vi "work1_Takeorder_and_Cook.vi"() -> ()   [LabVIEW 2026]
panel:
  out "Client Served":i32
  out "element":i32
  in  "stop":bool
  in  "Order ID":i32
  # "Producer Consumer Demo"
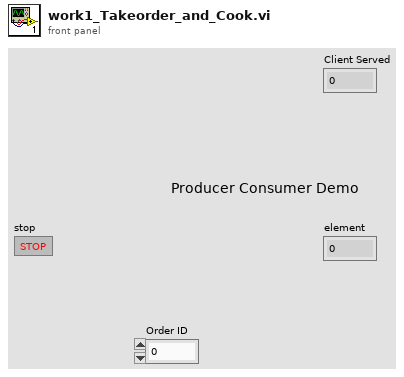
[diagram p1: front panel]
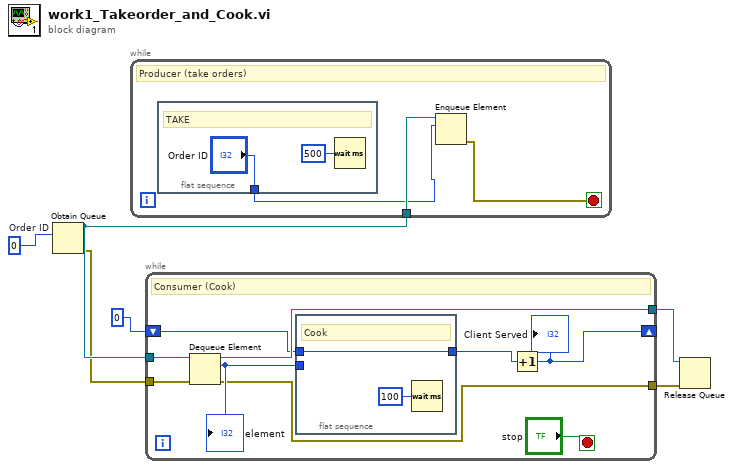
[diagram p0: block diagram]
diagram:
  w6 = 0  # Order ID
  n1 = Obtain Queue(element data type=w6) -> (queue out=w5:refnum<queue>, error out=w4:errorcluster)  [unwired: 4 in, 1 out]
  n2 = while {
    tunnel: w5 -> [w9]
    stop <- w7 stop-if-true
    # "Producer (take orders)"
    n3 = flat-sequence {
      tunnel: ["Order ID"] -> w8
      frame #0 {
        # "TAKE"
        n4 = Wait (ms)(milliseconds to wait=u32 500) -> ()  [unwired: 1 out]
      }
    }
    n5 = Enqueue Element(queue=w9, element=w8) -> (error out=w7:errorcluster)  [unwired: 2 in, 2 out]
  }
  n6 = while {
    tunnel: w5 -> [w20]
    tunnel: w4 -> [w19]
    tunnel: [w16] -> w3
    tunnel: [w15] -> w2
    shift-right: [w13] -> _
    shift-left: 0 -> [w14]
    stop <- "stop" stop-if-true
    # "Consumer (Cook)"
    n7 = Dequeue Element(queue=w20, error in (no error)=w19) -> (queue out=w16:refnum<queue>, element=w18:i32, error out=w15:errorcluster)  [unwired: 1 in, 1 out]
    "element" <- w18
    n8 = flat-sequence {
      tunnel: w18 -> [_]
      tunnel: w14 -> [w21]
      tunnel: [w21] -> w12
      frame #0 {
        # "Cook"
        n9 = Wait (ms)(milliseconds to wait=u32 100) -> ()  [unwired: 1 out]
      }
    }
    n10 = Increment(x=w12) -> (x+1=w13:i32)
    "Client Served" <- w13
  }
  n11 = Release Queue(queue=w3, error in (no error)=w2) -> ()  [unwired: 1 in, 3 out]
